vi "ReadCurrent.vi"(8 "error in (no error)":errorcluster, 11 "reference in":refnum<class "VdPhilipsMM-456.lvclass">) -> (0 "error out":errorcluster, 2 "Current":dbl, 3 "reference out":refnum<class "VdPhilipsMM-456.lvclass">)   [LabVIEW 2020, in "MulitMeters.lvlib" / "VdPhilipsMM-456.lvclass"]
uses:
  VdPhilipsMM-456.lvclass
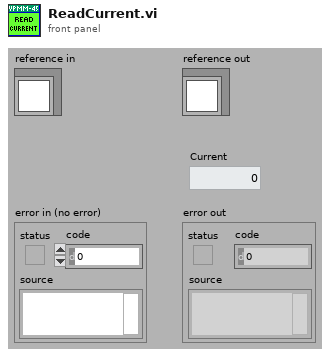
[diagram p1: front panel]
types:
  T1 = typedef "MulitMeters.lvlib/VdPhilipsMM-456.lvclass/ObjectAttributes.ctl" = cluster{"VISA Ref":refnum<visa-resource-name>}
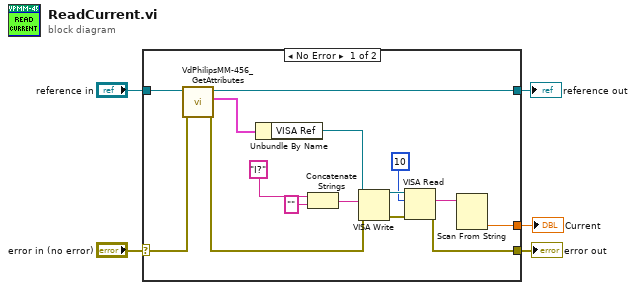
[diagram p0: block diagram]
diagram:
  n1 = case shown="No Error" "error in (no error)" {
    selector: "error in (no error)" -> [w20 w22]
    tunnel: [w11 w22] -> w4
    tunnel: [w17 w21] -> w2
    tunnel: "reference in" -> [w18 w21]
    tunnel: [w8 _] -> w1
    frame No Error {
      n2 = call "VdPhilipsMM-456_GetAttributes.vi"("error in (no error)"=w20, "reference in"=w18) -> ("error out"=w10:errorcluster, "Data"=w19:T1, "reference out"=w17:refnum<class "VdPhilipsMM-456.lvclass">)  [unwired: 6 in, 1 out]
      n3 = Unbundle By Name(w19) -> ("VISA Ref"=w16:refnum<visa-resource-name>)
      n4 = Concatenate Strings("I?", "" ("string")) -> (w14:string)
      n5 = VISA Write(VISA resource name=w16, write buffer=w14, error in (no error)=w10) -> (VISA resource name out=w12:refnum<visa-resource-name>, error out=w13:errorcluster)  [unwired: 1 out]
      n6 = VISA Read(VISA resource name=w12, byte count=u32 10, error in (no error)=w13) -> (read buffer=w9:string, error out=w11:errorcluster)  [unwired: 2 out]
      n7 = Scan From String(input string=w9) -> (output 1=w8:dbl)  [unwired: 4 in, 3 out]
    }
    frame Error {
    }
  }
  "error out" <- w4
  "reference out" <- w2
  "Current" <- w1
